vi "Run Streamed Request.vi"(0 "request":string, 1 "protocol version":string, 2 "Mcp-Method":string, 3 "Mcp-Name":string, 5 "id in":i32, 7 "events":refnum<queue>, 9 "cancelled":refnum<queue>, 11 "error in":errorcluster) -> (15 "error out":errorcluster)   [LabVIEW 2020, in "MCP Server.lvlib"]
doc: "Handles one streamed tools/call in the background (started by Start Streamed Request.vi, reentrant, never waited for). First resets Stream State.vi, so that no state left by an earlier stream applies, then calls Handle MCP Request.vi with the stream object {\"events\":..,\"cancelled\":..} so that Report Progress.vi and Cancel Requested.vi reach the queues of the MCP SSE Response through the request context. When it returns, sends the final JSON-RPC response as the last event \"data: <json>\" (for a modern request with all its result fields; resultType input_required when the tool asked the user) and the end marker (an empty string), which ends the stream.\n\nWhen the request was cancelled (the client closed the stream, Abort Stream ran, or a legacy notifications/cancelled named its id; all three are read after Handle MCP Request.vi has returned) no final response is sent, only the end marker. Afterwards it waits at most 5 s for the stream to take the last events and releases both queues.\n\nAll errors are cleared here: nobody waits for this VI, so an error must not open a dialog."
uses:
  MCP Server.lvlib
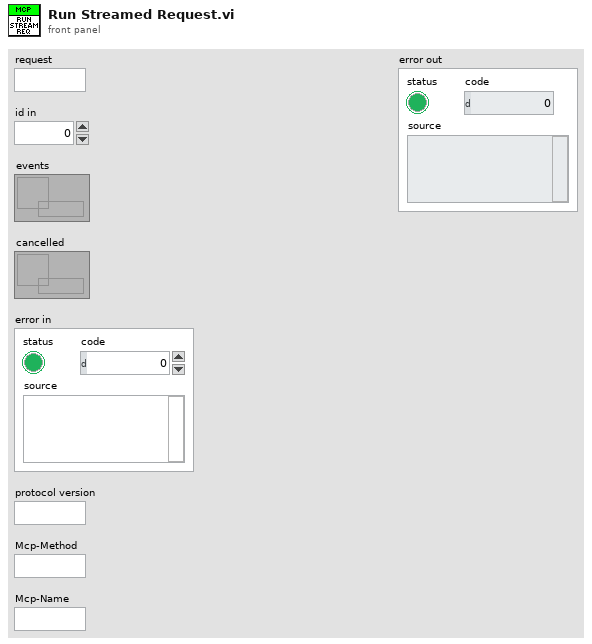
[diagram p1: front panel]
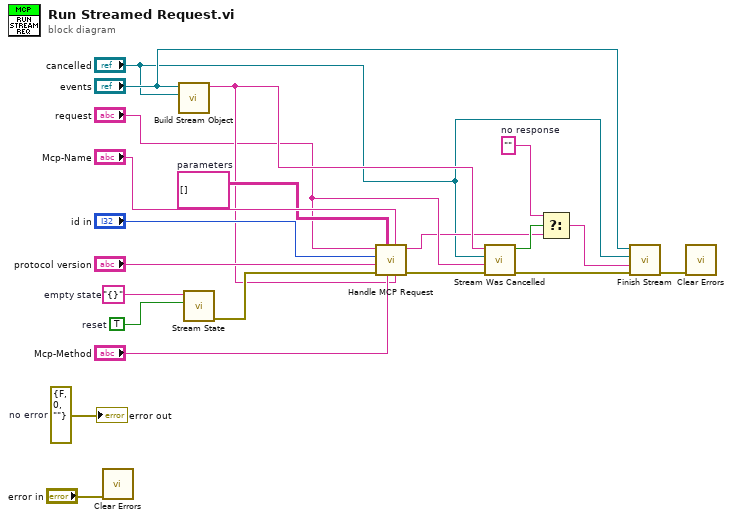
[diagram p0: block diagram]
diagram:
  w1 = errorcluster {"status"=FALSE, "code"=0, "source"=""}  # no error
  w9 = ""  # no response
  w20 = TRUE  # reset
  w19 = "{}"  # empty state
  w16 = string[][] []  # parameters
  n1 = call <vilib>:"Clear Errors.vi"("error in (no error)"="error in") -> ()  [unwired: 5 in, 2 out]
  n2 = call "Build Stream Object.vi"("cancelled"="cancelled", "events"="events") -> ("stream"=w12:string)  [unwired: 9 in]
  n3 = call "Stream State.vi"("set?"=w20, "state in"=w19) -> ("error out"=w15:errorcluster)  [unwired: 8 in, 1 out]
  n4 = call "Handle MCP Request.vi"("stream"=w12, "Mcp-Name"="Mcp-Name", "Mcp-Method"="Mcp-Method", "parameters"=w16, "error in"=w15, "protocol version"="protocol version", "id in"="id in", "request"="request") -> ("error out"=w10:errorcluster, "response"=w7:string)  [unwired: 1 in, 1 out]
  n5 = call "Stream Was Cancelled.vi"("error in"=w10, "request"="request", "cancelled"="cancelled", "stream"=w12) -> ("error out"=w3:errorcluster, "cancelled?"=w8:bool)  [unwired: 6 in]
  n6 = Select(t=w9, s=w8, f=w7) -> (s? t:f=w4:string)
  n7 = call "Finish Stream.vi"("error in"=w3, "response"=w4, "cancelled"="cancelled", "events"="events") -> ("error out"=w2:errorcluster)  [unwired: 7 in]
  n8 = call <vilib>:"Clear Errors.vi"("error in (no error)"=w2) -> ()  [unwired: 5 in, 2 out]
  "error out" <- w1
